vi "RemoteVI Check WS Encode Server Frame.vi"() -> (4 "labels":string[](array[string]), 6 "expected":string[](array[string]), 8 "actual":string[](array[string]), 10 "failures":i32)   [LabVIEW 2020]
doc: "Test support, generated by tests/caraya/build.py from tests/vectors/websocket.json (serverFrames) - do not edit. Calls RemoteVI WS Encode Server Frame.vi once per vector: payload is the vector's hex, or payloadLength zero bytes where the vector gives only the header; the frame is compared as lowercase hex, only its first bytes where the vector gives a header. Outputs, one element per vector: labels (the vector's name), expected (rendered from the vector), actual (the VI's result rendered the same way), and failures, the number of vectors whose expected and actual differ."
uses:
  source/RemoteVI.lvlib
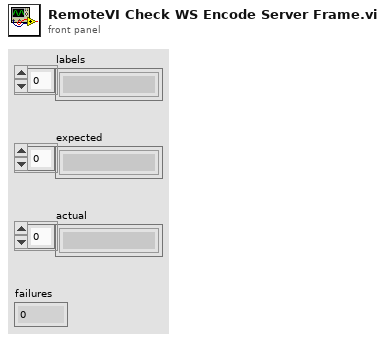
[diagram p1: front panel]
types:
  T1 = cluster{"name":string, "opcode":u8, "payload":string, "zeros":i32, "expect":string, "cmp":i32}[]
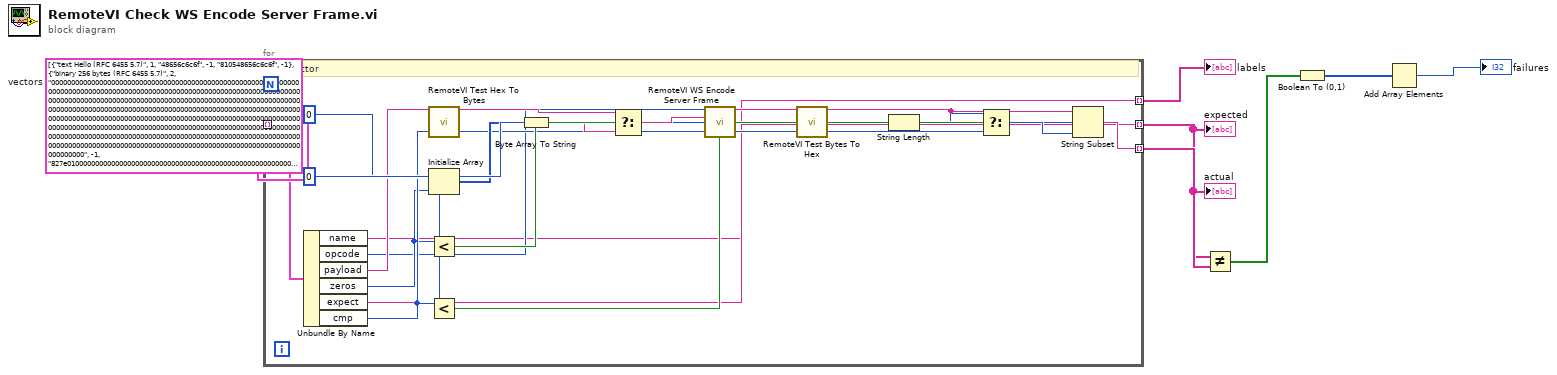
[diagram p0: block diagram]
diagram:
  w1 = T1 [{"name"="text Hello (RFC 6455 5.7)", "opcode"=1, "payload"="48656c6c6f", "zeros"=-1, "expect"="810548656c6c6f", "cmp"=-1}, {"name"="binary 256 bytes (RFC 6455 5.7)", "opcode"=2, "payload"="00000000000000000000000000000000000000000000000000000000000000000000000000000000000000000000000000000000000000000000000000000000000000000000000000000000000000000000000000000000000000000000000000000000000000000000000000000000000000000000000000000000000000000000000000000000000000000000000000000000000000000000000000000000000000000000000000000000000000000000000000000000000000000000000000000000000000000000000000000000000000000000000000000000000000000000000000000000000000000000000000000000000000000000000000000000", "zeros"=-1, "expect"="827e010000000000000000000000000000000000000000000000000000000000000000000000000000000000000000000000000000000000000000000000000000000000000000000000000000000000000000000000000000000000000000000000000000000000000000000000000000000000000000000000000000000000000000000000000000000000000000000000000000000000000000000000000000000000000000000000000000000000000000000000000000000000000000000000000000000000000000000000000000000000000000000000000000000000000000000000000000000000000000000000000000000000000000000000000000000000", "cmp"=-1}, {"name"="binary 65536 bytes header", "opcode"=2, "payload"="", "zeros"=65536, "expect"="827f0000000000010000", "cmp"=20}, {"name"="close 1000", "opcode"=8, "payload"="03e8", "zeros"=-1, "expect"="880203e8", "cmp"=-1}]  # vectors
  n1 = for {
    tunnel: w1 -> [w8] mode=indexing
    tunnel: [w9] -> w2 mode=indexing
    tunnel: [w13] -> w3 mode=indexing
    tunnel: [w27] -> w4 mode=indexing
    w19 = 0
    # "One vector"
    n2 = Unbundle By Name(w8) -> ("name"=w9:string, "opcode"=w10:u8, "payload"=w11:string, "zeros"=w12:i32, "expect"=w13:string, "cmp"=w14:i32)
    n3 = call "RemoteVI Test Hex To Bytes.vi"("hex"=w11) -> ("bytes"=w15:string)  [unwired: 14 in]
    n4 = Initialize Array(u8 0, w12) -> (w17:u8[])
    n5 = Less?(x=w12, y=w19) -> (x < y?=w20:bool)
    n6 = Less?(x=w14, y=w19) -> (x < y?=w25:bool)
    n7 = Byte Array To String(unsigned byte array=w17) -> (string=w18:string)
    n8 = Select(t=w15, s=w20, f=w18) -> (s? t:f=w21:string)
    n9 = call "RemoteVI WS Encode Server Frame.vi"("opcode"=w10, "payload"=w21) -> ("frame"=w22:string)  [unwired: 13 in]
    n10 = call "RemoteVI Test Bytes To Hex.vi"("bytes"=w22) -> ("hex"=w23:string)  [unwired: 14 in]
    n11 = String Length(string=w23) -> (length=w24:i32)
    n12 = Select(t=w24, s=w25, f=w14) -> (s? t:f=w26:i32)
    n13 = String Subset(string=w23, offset (0)=w19, length (rest)=w26) -> (substring=w27:string)
  }
  "labels" <- w2
  "expected" <- w3
  "actual" <- w4
  n14 = Not Equal?(x=w3, y=w4) -> (x != y?=w5:bool[])
  n15 = Boolean To (0,1)(Boolean=w5) -> (0, 1=w6:i16[])
  n16 = Add Array Elements(numeric array=w6) -> (sum=→"failures":i16)
